vi "Eval_MultiRes.vi"(8 "error in (no error)":errorcluster, 11 "muExpr in":refnum<class "mupExpr.lvclass">) -> (0 "error out":errorcluster, 2 "Results":dbl[](array[numeric]) format="%#_13g", 3 "muExpr out":refnum<class "mupExpr.lvclass">)   [LabVIEW 2015, in "mupExpr.lvclass"]
doc: "Evaluate all expressions and returns one result per expression.\n\nIf the variables are defined for bulk mode evaluation, only the first set (index 0) will be updated and evaluated."
uses:
  mupExpr.lvclass
  mupExpr.lvclass/mupExpr.ctl
  mupLib/mupCheckError.vi
  <vilib>/Utility/error.llb/Error Cluster From Error Code.vi
  mupLib/mupLib.lvlib
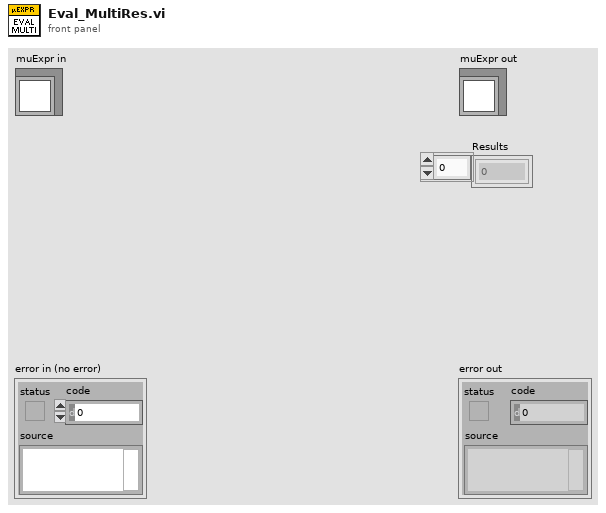
[diagram p1: front panel]
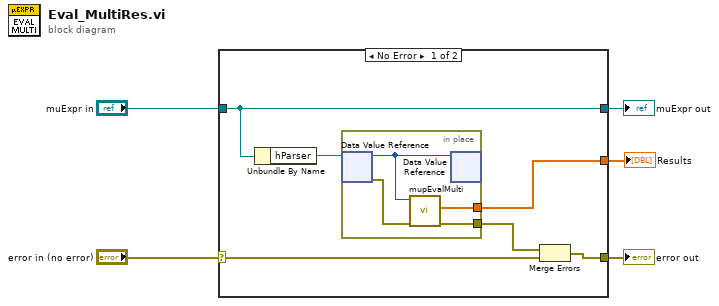
[diagram p0: block diagram]
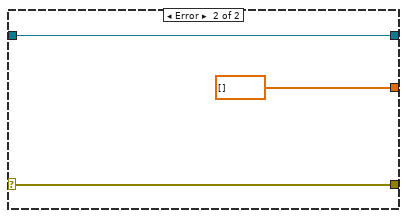
[diagram p2: hidden frame]
diagram:
  n1 = case shown="No Error" "error in (no error)" {
    selector: "error in (no error)" -> [w6 w18]
    tunnel: [w11 w18] -> w4
    tunnel: [w9 w17] -> w2
    tunnel: "muExpr in" -> [w9 w17]
    tunnel: [w8 dbl[] [] ("return type")] -> w1
    frame No Error {
      n2 = Unbundle By Name(w9) -> ("hParser"=w10:refnum<data-value>)
      n3 = in-place {
        in-place-border: [w15] -> w7
        in-place-border: [w13] -> w8
        n4 = in-place-dvr #1(w10) -> (w12:u64, w14:errorcluster)
        n5 = call "mupEvalMulti.vi"("error in (no error)"=w14, "hParser in"=w12) -> ("error out"=w15:errorcluster, "results"=w13:dbl[])  [unwired: 6 in, 2 out]
        n6 = in-place-dvr #1(w12) -> ()  [unwired: 2 out]
      }
      n7 = Merge Errors(w7, w6) -> (w11:errorcluster)
    }
    frame Error {
    }
  }
  "error out" <- w4
  "muExpr out" <- w2
  "Results" <- w1
